vi "UMLEditor_FixXmlData.vi"(10 "XmlTemplateIn":string, 11 "xmlIn":string) -> (3 "XML OUt":string)   [LabVIEW 2020]
panel:
  in  "Multicolumn Listbox":i32(listbox)
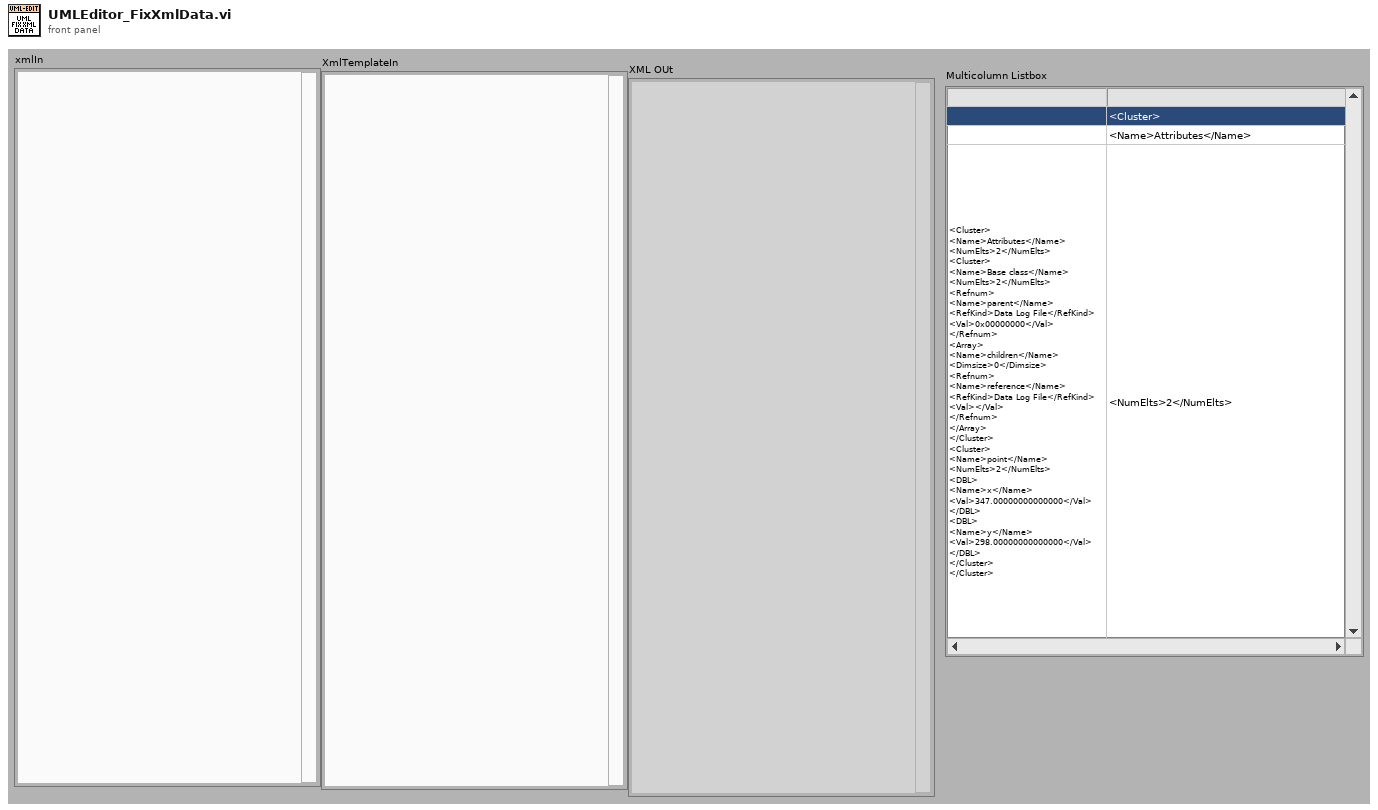
[diagram p1: front panel]
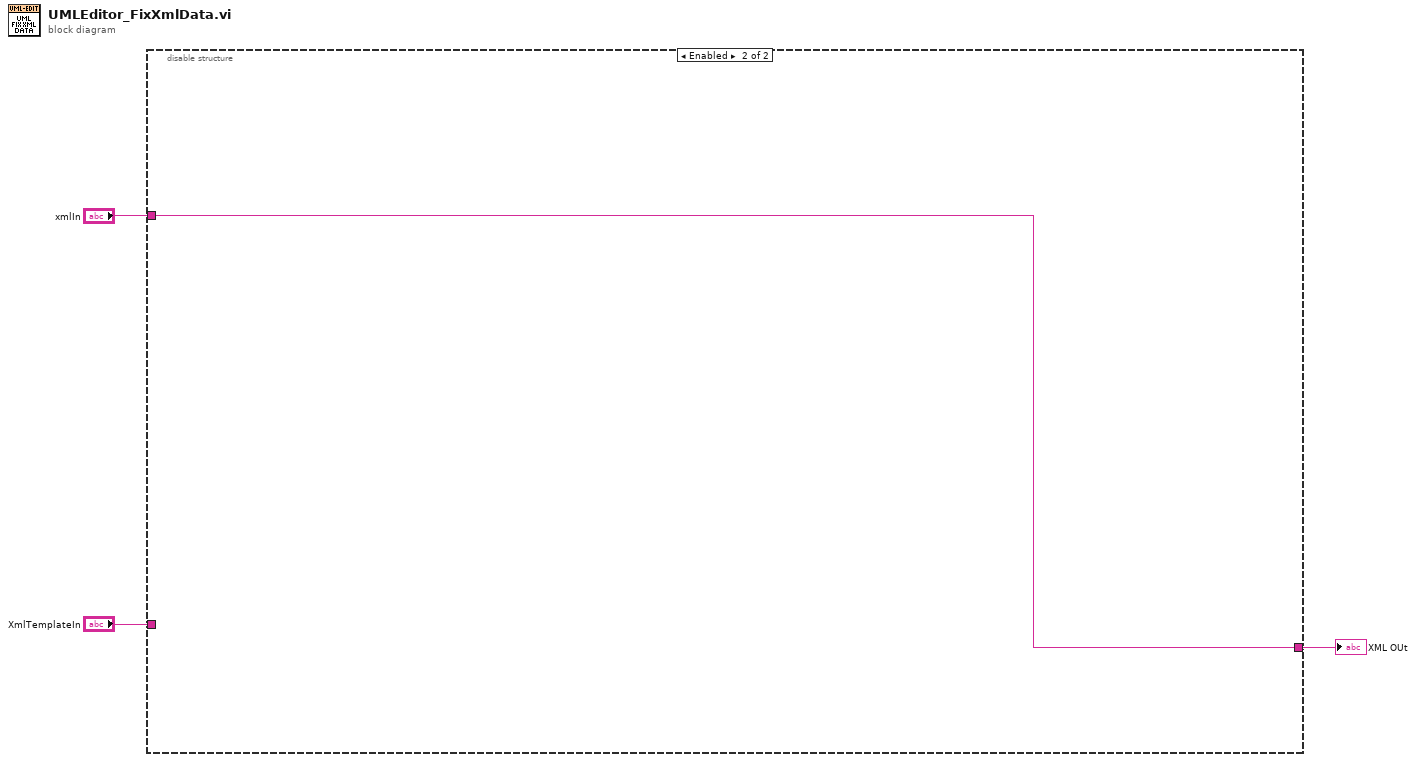
[diagram p0: block diagram]
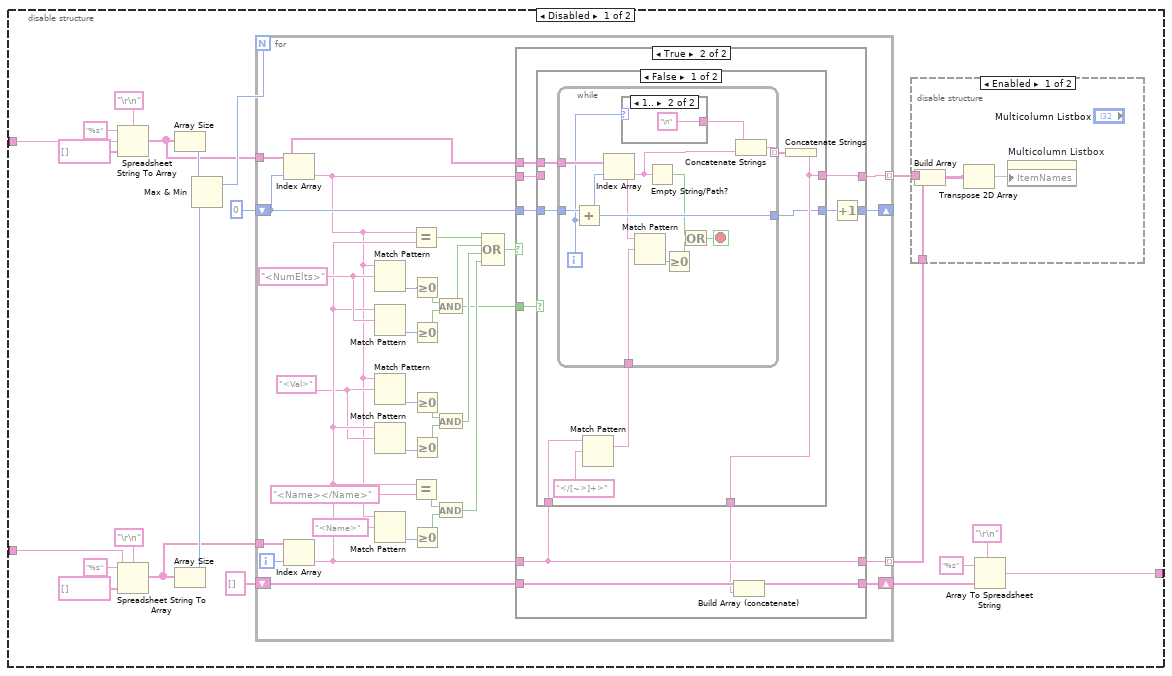
[diagram p2: hidden frame]
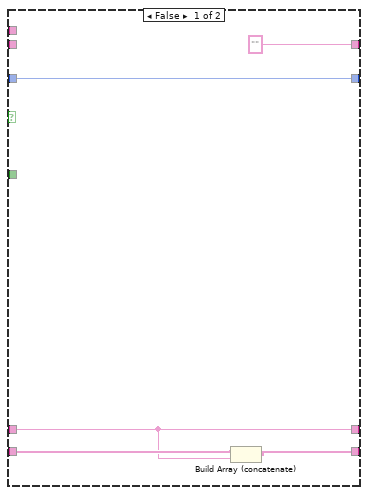
[diagram p4: hidden frame]
diagram:
  n1 = disable-structure shown="Enabled" {
    disable-tunnel: "xmlIn" -> [w24 w100]
    disable-tunnel: "XmlTemplateIn" -> [w17 _]
    disable-tunnel: [w4 w100] -> w1
    frame Disabled {
      n2 = Spreadsheet String To Array(delimiter (Tab)="\r\n", format string="%s", spreadsheet string=w24, array type (2D Dbl)=string[] []) -> (array=w13:string[])
      n3 = Spreadsheet String To Array(delimiter (Tab)="\r\n", format string="%s", spreadsheet string=w17, array type (2D Dbl)=string[] []) -> (array=w12:string[])
      n4 = Array Size(array=w13) -> (size(s)=w16:i32)
      n5 = Array Size(array=w12) -> (size(s)=w15:i32)
      n6 = Max & Min(x=w16, y=w15) -> (max(x,y)=w14:i32)  [unwired: 1 out]
      n7 = for {
        N: w14 -> [_]
        tunnel: w13 -> [w29]
        tunnel: w12 -> [w59]
        shift-right: [w53] -> _
        shift-left: 0 -> [w56]
        tunnel: [w55] -> w10 mode=indexing
        tunnel: [w54] -> w9 mode=indexing
        shift-right: [w32] -> w7
        shift-left: string[] [] -> [w31]
        i -> [w57]
        w39 = "<Val>" ("regular expression")
        w52 = "<NumElts>" ("regular expression")
        n8 = Index Array(array=w29, index=w56) -> (element=w33:string)
        n9 = Index Array(array=w59, index=w57) -> (element=w41:string)
        n10 = Match Pattern(string=w33, regular expression=w52) -> (offset past match=w51:i32)  [unwired: 4 out]
        n11 = Match Pattern(string=w41, regular expression=w52) -> (offset past match=w50:i32)  [unwired: 4 out]
        n12 = Match Pattern(string=w33, regular expression=w39) -> (offset past match=w44:i32)  [unwired: 4 out]
        n13 = Match Pattern(string=w41, regular expression=w39) -> (offset past match=w42:i32)  [unwired: 4 out]
        n14 = Match Pattern(string=w33, regular expression="<Name>") -> (offset past match=w37:i32)  [unwired: 4 out]
        n15 = Equal?(x=w33, y=w41) -> (x = y?=w58:bool)
        n16 = Equal?(x=w41, y="<Name></Name>") -> (x = y?=w36:bool)
        n17 = Greater Or Equal To 0?(x=w51) -> (x >= 0?=w49:bool)
        n18 = Greater Or Equal To 0?(x=w50) -> (x >= 0?=w48:bool)
        n19 = Greater Or Equal To 0?(x=w44) -> (x >= 0?=w45:bool)
        n20 = Greater Or Equal To 0?(x=w42) -> (x >= 0?=w46:bool)
        n21 = Greater Or Equal To 0?(x=w37) -> (x >= 0?=w35:bool)
        n22 = And(x=w49, y=w48) -> (x .and. y?=w30:bool)
        n23 = And(x=w45, y=w46) -> (x .and. y?=w43:bool)
        n24 = And(x=w36, y=w35) -> (x .and. y?=w34:bool)
        n25 = Compound Arithmetic op=OR(w58, w30, w43, w34) -> (w47:bool)
        n26 = case shown="True" w47 {
          tunnel: w56 -> [w64 w69]
          tunnel: w33 -> [_ w72]
          tunnel: w41 -> [w60 w73]
          tunnel: ["" w68] -> w55
          tunnel: [w60 w73] -> w54
          tunnel: [w64 w65] -> w53
          tunnel: [w61 w75] -> w32
          tunnel: w31 -> [w62 w74]
          tunnel: w30 -> [_ w70]
          tunnel: w29 -> [_ w67]
          frame False {
            n27 = Build Array (concatenate)(w62, w60) -> (w61:string[])
          }
          frame True {
            n28 = case shown="False" w70 {
              tunnel: w73 -> [w83 w99]
              tunnel: w72 -> [_ w98]
              tunnel: [w77 w99] -> w71
              tunnel: w69 -> [w80 w97]
              tunnel: [w76 w97] -> w66
              tunnel: [w77 w98] -> w68
              tunnel: w67 -> [w81 _]
              frame False {
                n29 = Match Pattern(string=w83, regular expression="</[~>]+>") -> (match substring=w79:string)  [unwired: 4 out]
                n30 = while {
                  tunnel: w81 -> [w95]
                  tunnel: w80 -> [w94]
                  tunnel: [w93] -> w76
                  tunnel: w79 -> [w92]
                  tunnel: [w86] -> w78 mode=indexing
                  i -> [w85]
                  stop <- w88 stop-if-true
                  n31 = Add(x=w94, y=w85) -> (x+y=w93:i32)
                  n32 = Index Array(array=w95, index=w93) -> (element=w87:string)
                  n33 = case shown="1.." w85 {
                    tunnel: [_ "\n" ("delimiter (Tab)")] -> w84
                    frame 0, Default {
                    }
                    frame 1.. {
                    }
                  }
                  n34 = Match Pattern(string=w87, regular expression=w92) -> (offset past match=w91:i32)  [unwired: 4 out]
                  n35 = Empty String/Path?(string/path=w87) -> (empty?=w89:bool)
                  n36 = Greater Or Equal To 0?(x=w91) -> (x >= 0?=w90:bool)
                  n37 = Or(x=w89, y=w90) -> (x .or. y?=w88:bool)
                  n38 = Concatenate Strings(w84, w87) -> (w86:string)
                }
                n39 = Concatenate Strings(w78) -> (w77:string)
              }
              frame True {
              }
            }
            n40 = Build Array (concatenate)(w74, w71) -> (w75:string[])
            n41 = Increment(x=w66) -> (x+1=w65:i32)
          }
        }
      }
      n42 = disable-structure shown="Enabled" {
        disable-tunnel: w10 -> [w28 _]
        disable-tunnel: w9 -> [w27 _]
        frame Enabled {
          n43 = Build Array(w28, w27) -> (w26:string[][])
          n44 = Transpose 2D Array(2D array=w26) -> (transposed array=w25:string[][])
          n45 = property on="Multicolumn Listbox" class="MCListbox (strict)"("ItemNames"=w25) -> ()  [unwired: 2 in, 2 out]
        }
        frame Disabled {
        }
      }
      n46 = Array To Spreadsheet String(delimiter (Tab)="\r\n", array=w7, 3:"%s" ("format string")) -> (spreadsheet string=w4:string)
    }
    frame Enabled {
    }
  }
  "XML OUt" <- w1
